vi "Set_Get_Filename_FVG.vi"(10 "Path":path, 11 "Enum":T1) -> (3 "Selected File path":path)   [LabVIEW 2021]
uses:
  Control/Set_Get.ctl
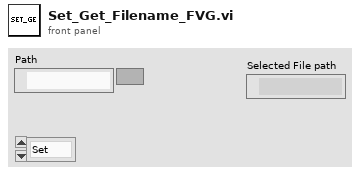
[diagram p1: front panel]
types:
  T1 = typedef "Set_Get.ctl" = enum16{"Set", "Get"}
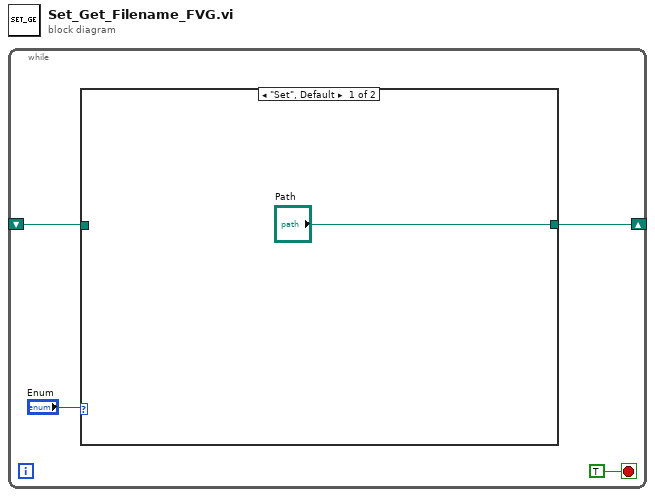
[diagram p0: block diagram]
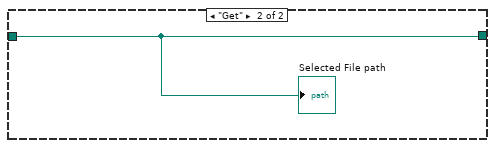
[diagram p2: hidden frame]
diagram:
  n1 = while {
    shift-right: [w3] -> _
    shift-left: _ -> [w2]
    stop <- TRUE stop-if-true
    n2 = case shown="\"Set\", Default" "Enum" {
      tunnel: ["Path" w6] -> w3
      tunnel: w2 -> [_ w6]
      frame "Set", Default {
      }
      frame "Get" {
        "Selected File path" <- w6
      }
    }
  }
